vi "Compare Folder Shot Files.vi"(8 "error in (no error)":errorcluster, 10 "Folder Shot File 2":path, 11 "Folder Shot File 1":path) -> (0 "error out":errorcluster, 3 "Folder Shot Results":T1)   [LabVIEW 2016, in "SLL File IO.lvlib"]
doc: "Compare two Folder Shot Files."
uses:
  SLL File IO.lvlib
  _Typedefs/Folder Shot Result.ctl
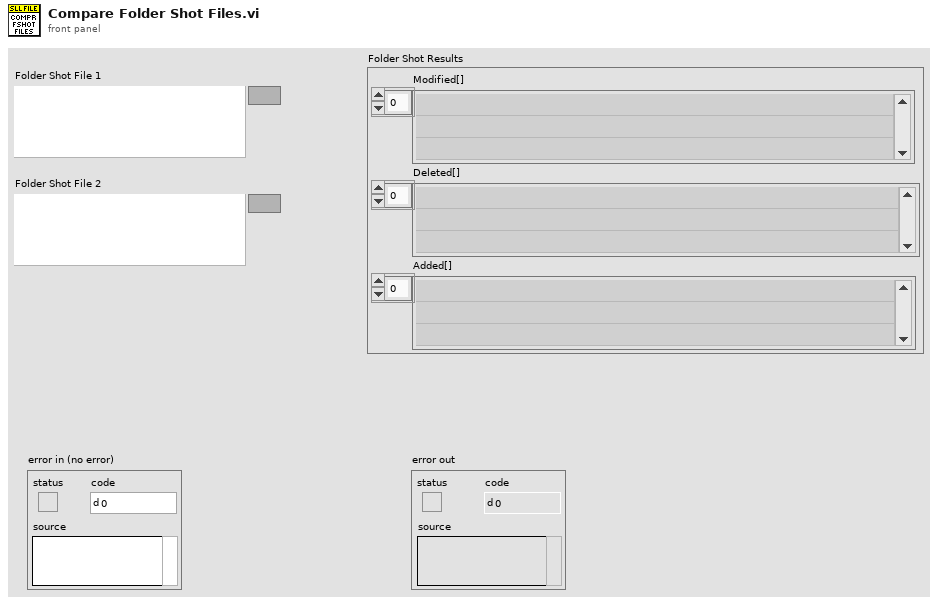
[diagram p1: front panel]
types:
  T1 = typedef "SLL File IO.lvlib/Folder Shot Result.ctl" = cluster{"Modified[]":path[], "Deleted[]":path[], "Added[]":path[]}
  T2 = typedef "SLL File IO.lvlib/Folder Shot Element.ctl" = cluster{"Abs.Path":path, "Relative Path":path, "MD5":string}
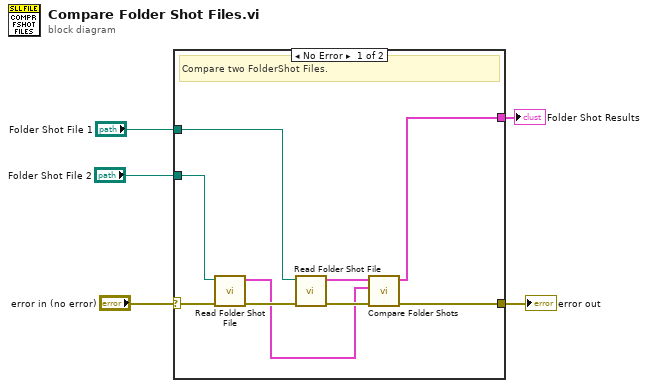
[diagram p0: block diagram]
diagram:
  n1 = case shown="No Error" "error in (no error)" {
    selector: "error in (no error)" -> [w14 w15]
    tunnel: [w9 w15] -> w4
    tunnel: "Folder Shot File 2" -> [w12 _]
    tunnel: "Folder Shot File 1" -> [w10 _]
    tunnel: [w6 _] -> w1
    frame No Error {
      # "Compare two FolderShot Files."
      n2 = call "Read Folder Shot File.vi"("error in (no error)"=w14, "Log Path"=w12) -> ("error out"=w13:errorcluster, "Folder Shot"=w7:T2[])  [unwired: 8 in]
      n3 = call "Read Folder Shot File.vi"("error in (no error)"=w13, "Log Path"=w10) -> ("error out"=w11:errorcluster, "Folder Shot"=w8:T2[])  [unwired: 8 in]
      n4 = call "Compare Folder Shots.vi"("error in (no error)"=w11, "Folder Shot 2"=w7, "Folder Shot 1"=w8) -> ("error out"=w9:errorcluster, "Folder Shot Results"=w6:T1)  [unwired: 7 in]
    }
    frame Error {
    }
  }
  "error out" <- w4
  "Folder Shot Results" <- w1
